vi "TEST_Menu.vi"() -> ()   [LabVIEW 2021, in "Menu.lvlib" / "Menu.lvclass"]
uses:
  Menu.lvclass
  <vilib>/Utility/miscctls.llb/LVMenuShortCut.ctl
  MenuSelection.ctl
  Picture2D/src/Color/Color.lvclass
  Picture2D/src/2DPictureControl/2DPictureControl.lvclass
  <vilib>/Utility/miscctls.llb/LVPointTypeDef.ctl
  91be992c-c2ba-4221-a176-dbd6ab68e1f9.vi
  Picture2D/src/Picture/Image.lvclass
  C:/GitHub/Picture2D/src/IDrawable/IDrawable.lvclass
  SetBackgroundColor.vi
  SetBorderColor.vi
  SetHiliteColor.vi
  SetHiliteTextColor.vi
  SetTextColor.vi
  <vilib>/ErrorRing/Error Ring.xnode
panel:
  out "enabled":bool
  out "2D Picture out":picture
  in  "Color Theme":enum16{"LabVIEW", "Dark"}(ring)
  out "item name":string
  out "submenu tags":string[](array[string])
  out "checked":bool
  out "short cut":T1
  out "2D Picture":picture
  out "ItemPath":string
  out "ItemTag":string
  out "error out":errorcluster
  out "item tags out":string[](array[string])
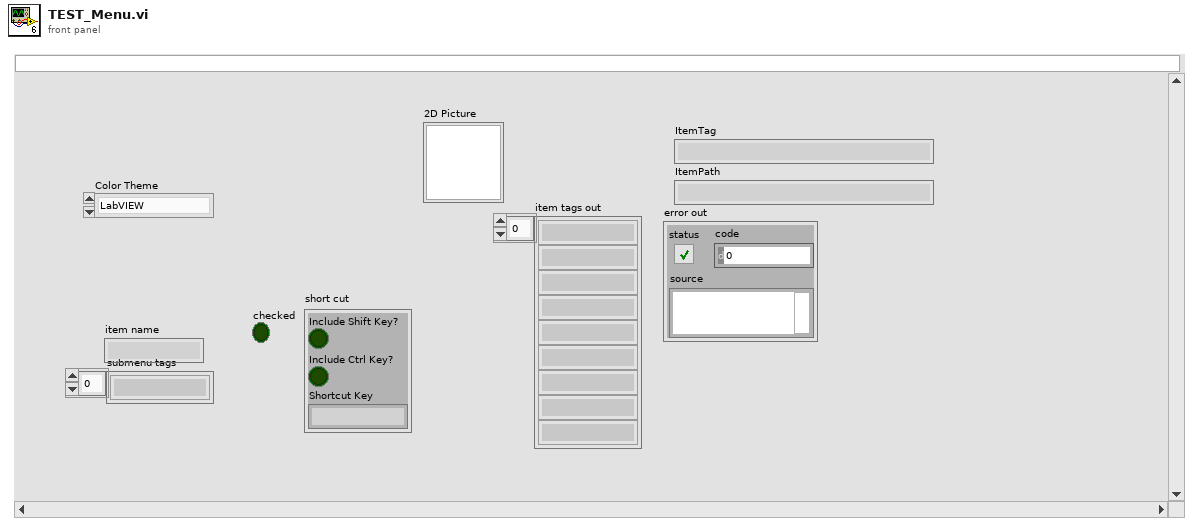
[diagram p1: front panel]
types:
  T1 = typedef "LVMenuShortCut.ctl" = cluster{"Include Shift Key?":bool, "Include Ctrl Key?":bool, "Shortcut Key":string}
  T2 = enum16{"Init Menu", "Init Menu Icon", "Execute", "Close"}
  T3 = enum16{"Init Menu", "Init Menu Icon", "Execute", "Close"}[]
  T4 = typedef "LVPointTypeDef.ctl" = cluster{"Horizontal":i16, "Vertical":i16}
  T5 = typedef "LVBoundsTypeDef.ctl" = cluster{"Width":u32, "Height":u32}
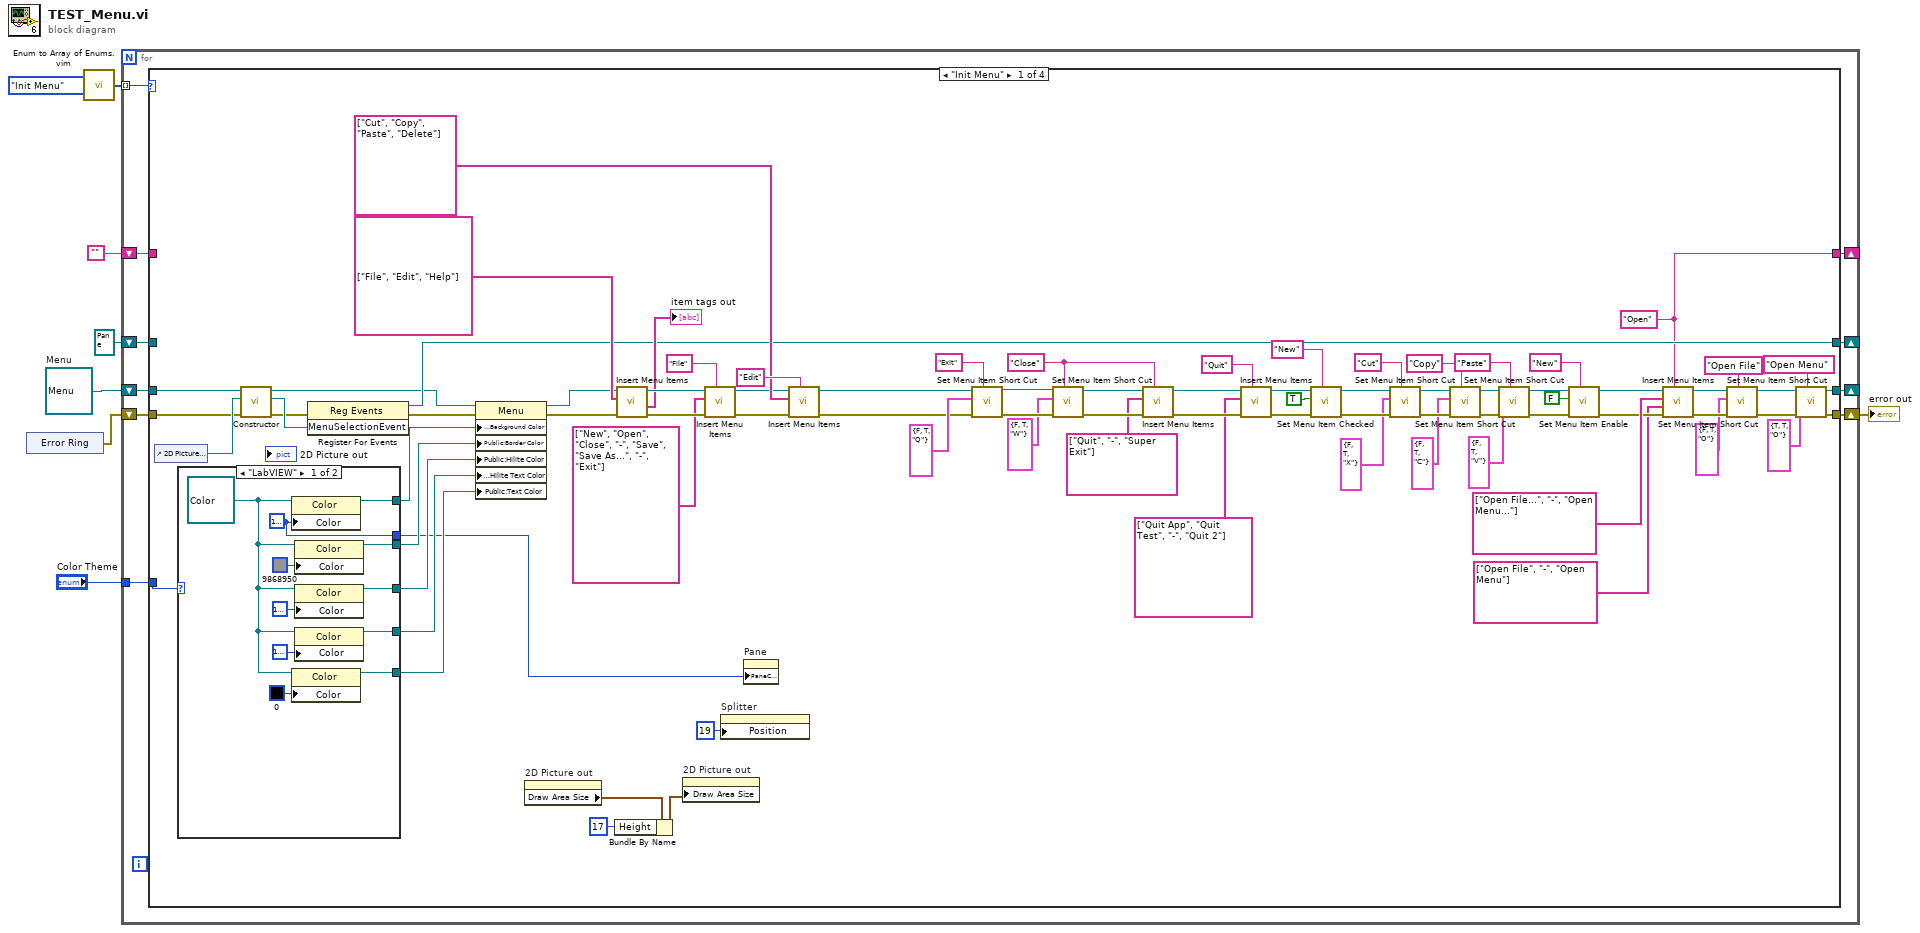
[diagram p0: block diagram]
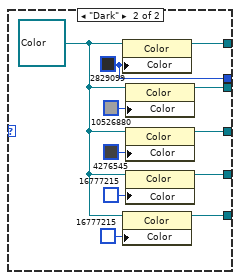
[diagram p2: hidden frame]
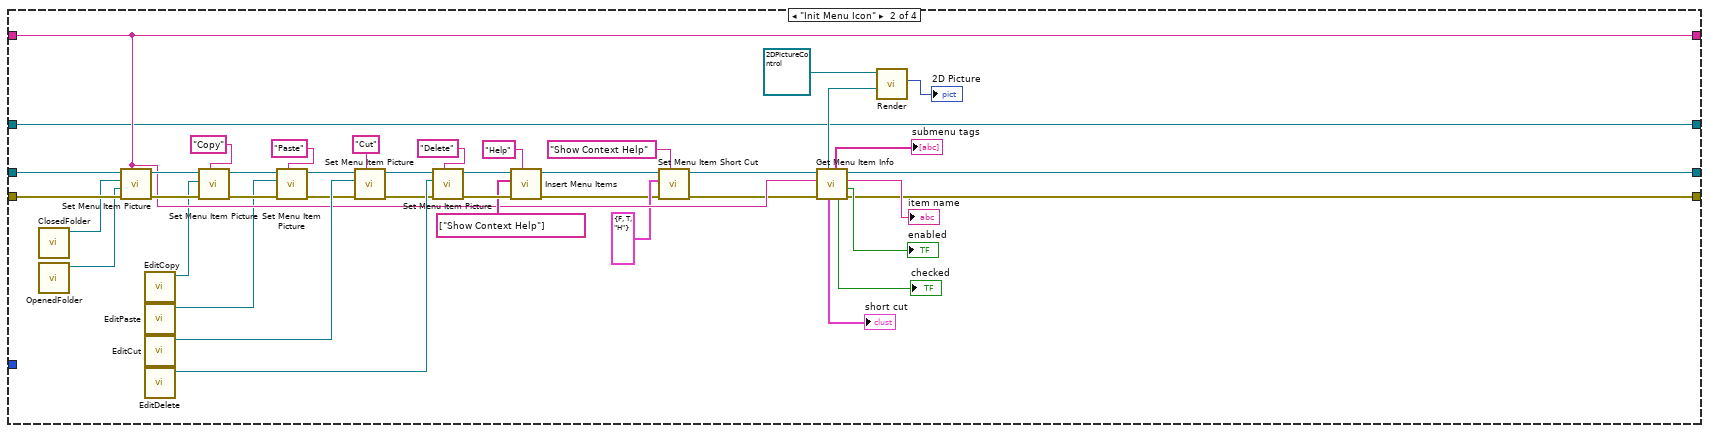
[diagram p3: hidden frame]
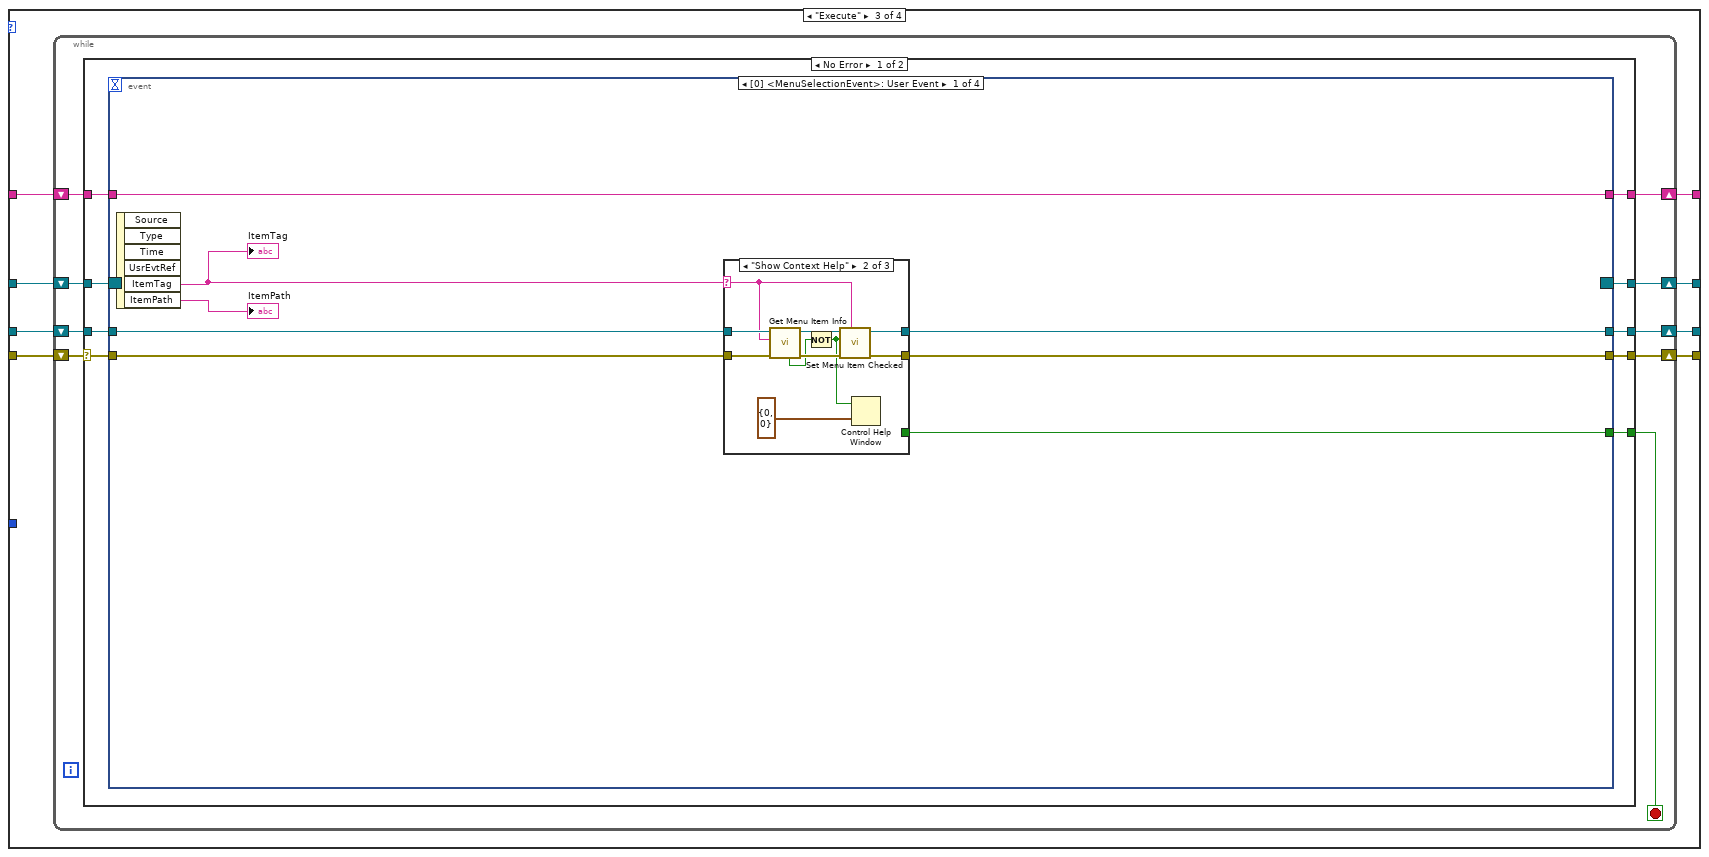
[diagram p4: hidden frame]
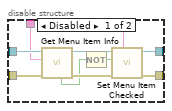
[diagram p6: hidden frame]
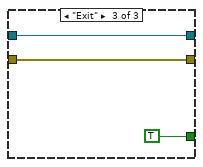
[diagram p7: hidden frame]
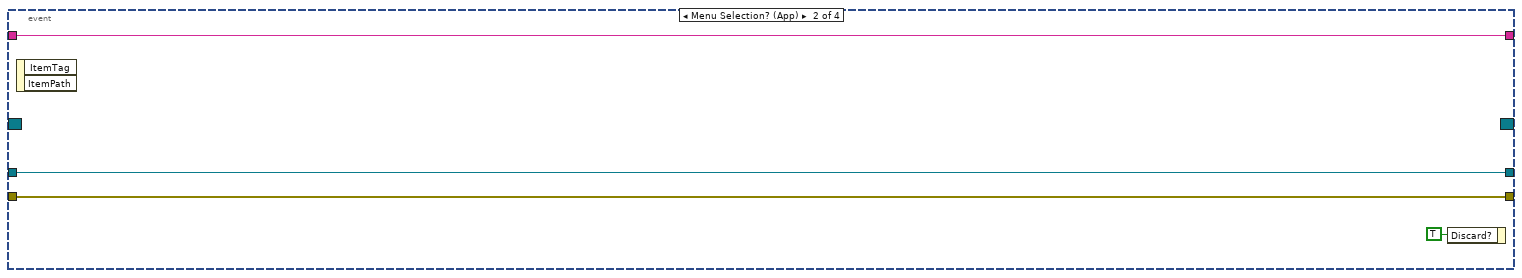
[diagram p8: hidden frame]
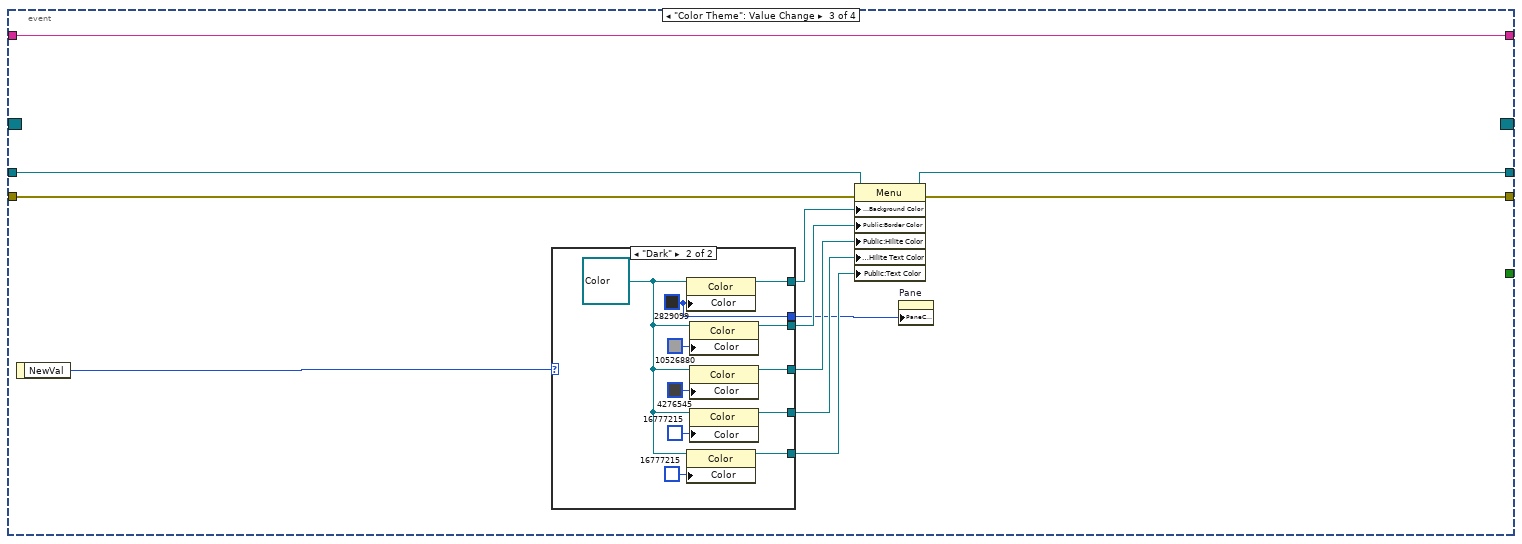
[diagram p9: hidden frame]
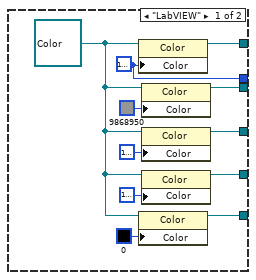
[diagram p10: hidden frame]
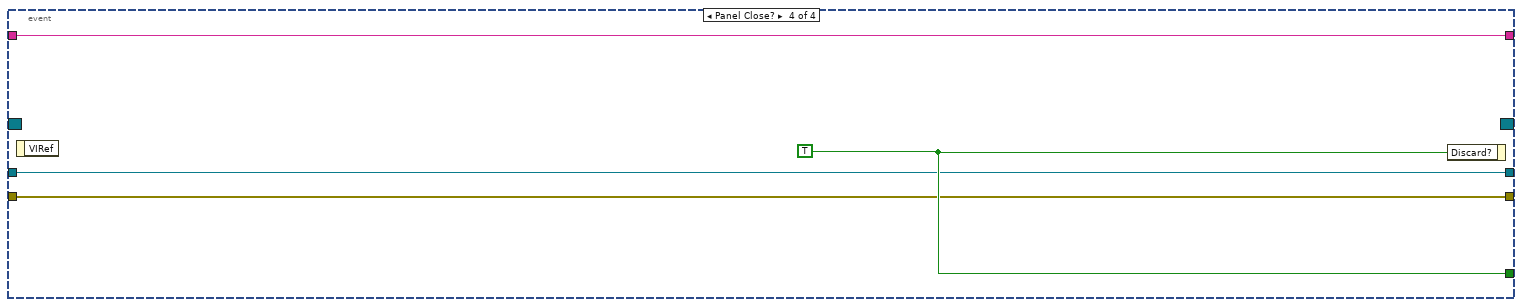
[diagram p11: hidden frame]
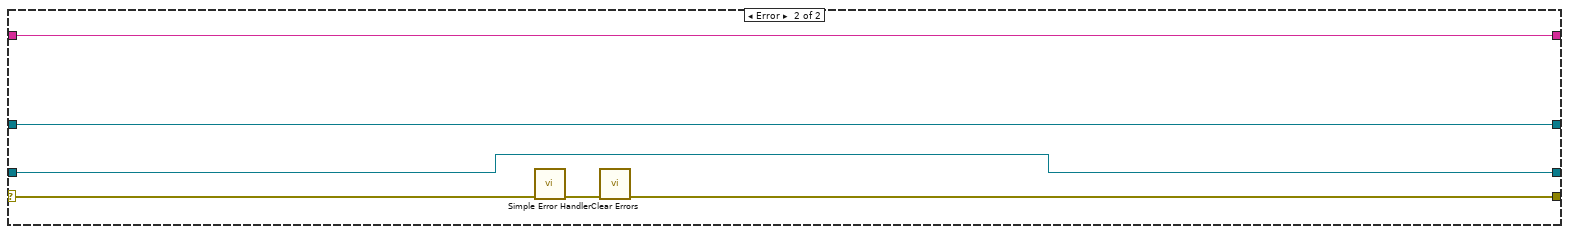
[diagram p12: hidden frame]
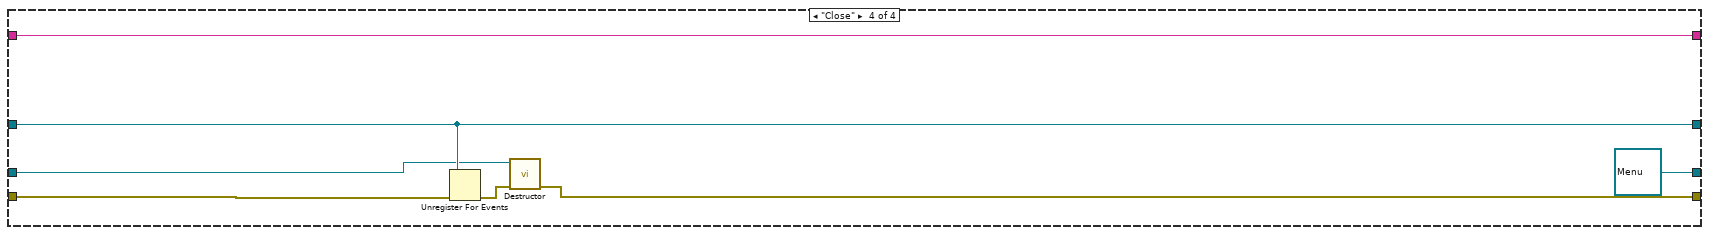
[diagram p13: hidden frame]
diagram:
  w8 = refnum<class "Menu.lvclass"> refnum  # Menu
  n1 = xnode "Error Ring"() -> ("error out"=w4:errorcluster)
  n2 = call "Enum to Array of Enums.vim"("enum"=T2."Init Menu") -> ("array of enums"=w5:T3)
  n3 = for {
    tunnel: "Color Theme" -> [w16]
    shift-right: [w15] -> _
    shift-left: w8 -> [w18]
    tunnel: w5 -> [w12] mode=indexing
    shift-right: [w14] -> w3
    shift-left: w4 -> [w13]
    shift-right: [w17] -> _
    shift-left: refnum<event-registration> refnum ("Event Registration Refnum") -> [w9]
    shift-right: [w11] -> _
    shift-left: "" -> [w10]
    n4 = case shown="\"Init Menu\"" w12 {
      tunnel: w18 -> [w99 w134 w169 w278]
      tunnel: [w74 w135 w170 w280] -> w17
      tunnel: [w68 w136 w164 w276] -> w11
      tunnel: w16 -> [w40 _ _ _]
      tunnel: [w33 w137 w168 refnum<class "Menu.lvclass"> refnum ("Menu")] -> w15
      tunnel: [w32 w138 w167 w279] -> w14
      tunnel: w13 -> [w26 w133 w166 w275]
      tunnel: w10 -> [_ w136 w165 w276]
      tunnel: w9 -> [_ w135 w171 w280]
      frame "Init Menu" {
        w68 = "Open" ("item tag")
        w81 = "Close" ("item tag")
        n5 = control-ref of="2D Picture out"() -> (w75:refnum<vi>)
        n6 = case shown="\"LabVIEW\"" w40 {
          tunnel: [w110 w121] -> w45
          tunnel: [w108 w119] -> w44
          tunnel: [w107 w118] -> w43
          tunnel: [w106 w117] -> w42
          tunnel: [w105 w116] -> w41
          tunnel: [w100 w111] -> w39
          frame "LabVIEW" {
            w100 = u32 16777238 ("Color")
            w109 = refnum<class "Color.lvclass"> refnum ("Background Color")
            n7 = property class="Color"(reference=w109, "Color"=w100) -> (reference out=w110:refnum<class "Color.lvclass">)  [unwired: 1 in, 1 out]
            n8 = property class="Color"(reference=w109, "Color"=u32 0) -> (reference out=w105:refnum<class "Color.lvclass">)  [unwired: 1 in, 1 out]
            n9 = property class="Color"(reference=w109, "Color"=u32 9868950) -> (reference out=w108:refnum<class "Color.lvclass">)  [unwired: 1 in, 1 out]
            n10 = property class="Color"(reference=w109, "Color"=u32 16777224) -> (reference out=w107:refnum<class "Color.lvclass">)  [unwired: 1 in, 1 out]
            n11 = property class="Color"(reference=w109, "Color"=u32 16777226) -> (reference out=w106:refnum<class "Color.lvclass">)  [unwired: 1 in, 1 out]
          }
          frame "Dark" {
            w111 = u32 2829099 ("Color")
            w120 = refnum<class "Color.lvclass"> refnum ("Background Color")
            n12 = property class="Color"(reference=w120, "Color"=w111) -> (reference out=w121:refnum<class "Color.lvclass">)  [unwired: 1 in, 1 out]
            n13 = property class="Color"(reference=w120, "Color"=u32 16777215) -> (reference out=w116:refnum<class "Color.lvclass">)  [unwired: 1 in, 1 out]
            n14 = property class="Color"(reference=w120, "Color"=u32 10526880) -> (reference out=w119:refnum<class "Color.lvclass">)  [unwired: 1 in, 1 out]
            n15 = property class="Color"(reference=w120, "Color"=u32 4276545) -> (reference out=w118:refnum<class "Color.lvclass">)  [unwired: 1 in, 1 out]
            n16 = property class="Color"(reference=w120, "Color"=u32 16777215) -> (reference out=w117:refnum<class "Color.lvclass">)  [unwired: 1 in, 1 out]
          }
        }
        n17 = call "Constructor.vi"("error in (no error)"=w26, "PictRef"=w75, "Menu in"=w99) -> ("error out"=w90:errorcluster, "MenuSelectionEvent"=w92:refnum<user-event>, "Menu out"=w47:refnum<class "Menu.lvclass">)  [unwired: 6 in]
        n18 = register-events(error in=w90, w92) -> (reference out=w74:refnum<event-registration>, error out=w91:errorcluster)  [unwired: 1 in]
        n19 = property class="Menu"(reference=w47, error in=w91, "Public:Background Color"=w45, "Public:Border Color"=w44, "Public:Hilite Color"=w43, "Public:Hilite Text Color"=w42, "Public:Text Color"=w41) -> (reference out=w46:refnum<class "Menu.lvclass">, error out=w48:errorcluster)
        n20 = property on="2D Picture out" class="Pict"() -> ("Draw Area Size"=w24:T5)  [unwired: 2 in, 2 out]
        n21 = Bundle By Name(cluster=w24, "Height"=u32 17) -> (w23:T5)
        n22 = call "Insert Menu Items.vi"("error in (no error)"=w48, "item names"=string[] ["File", "Edit", "Help"], "Menu in"=w46) -> ("error out"=w96:errorcluster, "item tags out"=→"item tags out":string[], "Menu out"=w97:refnum<class "Menu.lvclass">)  [unwired: 6 in]
        n23 = property on="2D Picture out" class="Pict"("Draw Area Size"=w23) -> ()  [unwired: 2 in, 2 out]
        n24 = call "Insert Menu Items.vi"("menu tag"="File", "error in (no error)"=w96, "item names"=string[] ["New", "Open", "Close", "-", "Save", "Save As...", "-", "Exit"], "Menu in"=w97) -> ("error out"=w49:errorcluster, "Menu out"=w50:refnum<class "Menu.lvclass">)  [unwired: 5 in, 1 out]
        n25 = property on="Splitter" class="Splitter"("Position"=19 ("Splitter Position")) -> ()  [unwired: 2 in, 2 out]
        n26 = property on="Pane" class="Pane"("PaneColor"=w39) -> ()  [unwired: 2 in, 2 out]
        n27 = call "Insert Menu Items.vi"("menu tag"="Edit", "error in (no error)"=w49, "item names"=string[] ["Cut", "Copy", "Paste", "Delete"], "Menu in"=w50) -> ("error out"=w21:errorcluster, "Menu out"=w20:refnum<class "Menu.lvclass">)  [unwired: 5 in, 1 out]
        n28 = call "Set Menu Item Short Cut.vi"("item tag"="Exit", "error in (no error)"=w21, "short cut"=T1 {"Include Shift Key?"=FALSE, "Include Ctrl Key?"=TRUE, "Shortcut Key"="Q"}, "Menu in"=w20) -> ("error out"=w86:errorcluster, "Menu out"=w85:refnum<class "Menu.lvclass">)  [unwired: 6 in]
        n29 = call "Set Menu Item Short Cut.vi"("item tag"=w81, "error in (no error)"=w86, "short cut"=T1 {"Include Shift Key?"=FALSE, "Include Ctrl Key?"=TRUE, "Shortcut Key"="W"}, "Menu in"=w85) -> ("error out"=w82:errorcluster, "Menu out"=w83:refnum<class "Menu.lvclass">)  [unwired: 6 in]
        n30 = call "Insert Menu Items.vi"("menu tag"=w81, "error in (no error)"=w82, "item names"=string[] ["Quit", "-", "Super Exit"], "Menu in"=w83) -> ("error out"=w78:errorcluster, "Menu out"=w77:refnum<class "Menu.lvclass">)  [unwired: 5 in, 1 out]
        n31 = call "Insert Menu Items.vi"("menu tag"="Quit", "error in (no error)"=w78, "item names"=string[] ["Quit App", "Quit Test", "-", "Quit 2"], "Menu in"=w77) -> ("error out"=w72:errorcluster, "Menu out"=w73:refnum<class "Menu.lvclass">)  [unwired: 5 in, 1 out]
        n32 = call "Set Menu Item Checked.vi"("item tag"="New", "error in (no error)"=w72, "checked"=TRUE, "Menu in"=w73) -> ("error out"=w66:errorcluster, "Menu out"=w67:refnum<class "Menu.lvclass">)  [unwired: 6 in]
        n33 = call "Set Menu Item Short Cut.vi"("item tag"="Cut", "error in (no error)"=w66, "short cut"=T1 {"Include Shift Key?"=FALSE, "Include Ctrl Key?"=TRUE, "Shortcut Key"="X"}, "Menu in"=w67) -> ("error out"=w63:errorcluster, "Menu out"=w62:refnum<class "Menu.lvclass">)  [unwired: 6 in]
        n34 = call "Set Menu Item Short Cut.vi"("item tag"="Copy", "error in (no error)"=w63, "short cut"=T1 {"Include Shift Key?"=FALSE, "Include Ctrl Key?"=TRUE, "Shortcut Key"="C"}, "Menu in"=w62) -> ("error out"=w65:errorcluster, "Menu out"=w64:refnum<class "Menu.lvclass">)  [unwired: 6 in]
        n35 = call "Set Menu Item Short Cut.vi"("item tag"="Paste", "error in (no error)"=w65, "short cut"=T1 {"Include Shift Key?"=FALSE, "Include Ctrl Key?"=TRUE, "Shortcut Key"="V"}, "Menu in"=w64) -> ("error out"=w56:errorcluster, "Menu out"=w54:refnum<class "Menu.lvclass">)  [unwired: 6 in]
        n36 = call "Set Menu Item Enable.vi"("item tag"="New", "error in (no error)"=w56, "enabled"=FALSE, "Menu in"=w54) -> ("error out"=w55:errorcluster, "Menu out"=w53:refnum<class "Menu.lvclass">)  [unwired: 6 in]
        n37 = call "Insert Menu Items.vi"("menu tag"=w68, "error in (no error)"=w55, "item tags"=string[] ["Open File", "-", "Open Menu"] ("item names"), "item names"=string[] ["Open File...", "-", "Open Menu..."], "Menu in"=w53) -> ("error out"=w36:errorcluster, "Menu out"=w37:refnum<class "Menu.lvclass">)  [unwired: 4 in, 1 out]
        n38 = call "Set Menu Item Short Cut.vi"("item tag"="Open File", "error in (no error)"=w36, "short cut"=T1 {"Include Shift Key?"=FALSE, "Include Ctrl Key?"=TRUE, "Shortcut Key"="O"}, "Menu in"=w37) -> ("error out"=w35:errorcluster, "Menu out"=w34:refnum<class "Menu.lvclass">)  [unwired: 6 in]
        n39 = call "Set Menu Item Short Cut.vi"("item tag"="Open Menu", "error in (no error)"=w35, "short cut"=T1 {"Include Shift Key?"=TRUE, "Include Ctrl Key?"=TRUE, "Shortcut Key"="O"}, "Menu in"=w34) -> ("error out"=w32:errorcluster, "Menu out"=w33:refnum<class "Menu.lvclass">)  [unwired: 6 in]
      }
      frame "Init Menu Icon" {
        n40 = call "ClosedFolder.vi"() -> ("Image out"=w123:refnum<class "Image.lvclass">)  [unwired: 11 in]
        n41 = call "OpenedFolder.vi"() -> ("Image out"=w122:refnum<class "Image.lvclass">)  [unwired: 11 in]
        n42 = call "Set Menu Item Picture.vi"("item tag"=w136, "error in (no error)"=w133, "Hilite Picture"=w122, "Picture"=w123, "Menu in"=w134) -> ("error out"=w153:errorcluster, "Menu out"=w152:refnum<class "Menu.lvclass">)  [unwired: 5 in]
        n43 = call "EditCopy.vi"() -> ("Image out"=w125:refnum<class "Image.lvclass">)  [unwired: 11 in]
        n44 = call "EditPaste.vi"() -> ("Image out"=w124:refnum<class "Image.lvclass">)  [unwired: 11 in]
        n45 = call "EditCut.vi"() -> ("Image out"=w162:refnum<class "Image.lvclass">)  [unwired: 11 in]
        n46 = call "EditDelete.vi"() -> ("Image out"=w163:refnum<class "Image.lvclass">)  [unwired: 11 in]
        n47 = call "Set Menu Item Picture.vi"("item tag"="Copy", "error in (no error)"=w153, "Picture"=w125, "Menu in"=w152) -> ("error out"=w155:errorcluster, "Menu out"=w154:refnum<class "Menu.lvclass">)  [unwired: 6 in]
        n48 = call "Set Menu Item Picture.vi"("item tag"="Paste", "error in (no error)"=w155, "Picture"=w124, "Menu in"=w154) -> ("error out"=w157:errorcluster, "Menu out"=w156:refnum<class "Menu.lvclass">)  [unwired: 6 in]
        n49 = call "Set Menu Item Picture.vi"("item tag"="Cut", "error in (no error)"=w157, "Picture"=w162, "Menu in"=w156) -> ("error out"=w159:errorcluster, "Menu out"=w158:refnum<class "Menu.lvclass">)  [unwired: 6 in]
        n50 = call "Set Menu Item Picture.vi"("item tag"="Delete", "error in (no error)"=w159, "Picture"=w163, "Menu in"=w158) -> ("error out"=w161:errorcluster, "Menu out"=w160:refnum<class "Menu.lvclass">)  [unwired: 6 in]
        n51 = call "Insert Menu Items.vi"("menu tag"="Help", "error in (no error)"=w161, "item names"=string[] ["Show Context Help"], "Menu in"=w160) -> ("error out"=w131:errorcluster, "Menu out"=w129:refnum<class "Menu.lvclass">)  [unwired: 5 in, 1 out]
        n52 = call "Set Menu Item Short Cut.vi"("item tag"="Show Context Help", "error in (no error)"=w131, "short cut"=T1 {"Include Shift Key?"=FALSE, "Include Ctrl Key?"=TRUE, "Shortcut Key"="H"}, "Menu in"=w129) -> ("error out"=w130:errorcluster, "Menu out"=w128:refnum<class "Menu.lvclass">)  [unwired: 6 in]
        n53 = call "Get Menu Item Info.vi"("error in (no error)"=w130, "item tag"=w136, "Menu in"=w128) -> ("error out"=w138:errorcluster, "enabled"=→"enabled":bool, "item name"=→"item name":string, "Menu out"=w137:refnum<class "Menu.lvclass">, "checked"=→"checked":bool, "submenu tags"=→"submenu tags":string[], "short cut"=→"short cut":T1, "Picture"=w140:refnum<class "Image.lvclass">)  [unwired: 1 in]
        n54 = call-dynamic "Render.vi"("IDrawable"=w140, "2DPictureControl in"=refnum<class "2DPictureControl.lvclass"> refnum) -> ("2D Picture out"=→"2D Picture":picture)  [unwired: 7 in, 2 out]
      }
      frame "Execute" {
        n55 = while {
          shift-right: [w178] -> w167
          shift-left: w166 -> [w179]
          shift-right: [w175] -> w170
          shift-left: w171 -> [w180]
          shift-right: [w176] -> w168
          shift-left: w169 -> [w177]
          shift-right: [w172] -> w164
          shift-left: w165 -> [w173]
          stop <- w174 stop-if-true
          n56 = case shown="No Error" w179 {
            selector: w179 -> [w188 w274]
            tunnel: w180 -> [w189 w273]
            tunnel: [w187 w270] -> w178
            tunnel: w177 -> [w186 w272]
            tunnel: [w185 w272] -> w176
            tunnel: [w184 w273] -> w175
            tunnel: [w183 _] -> w174
            tunnel: w173 -> [w182 w269]
            tunnel: [w181 w269] -> w172
            frame No Error {
              n57 = event shown="[0] <MenuSelectionEvent>: User Event" {
                selector: w189 -> [_ _ _ _]
                dyn-events: [_ _ _ _] -> w184
                timeout: _ -> [_ _ _ _]
                tunnel: [w192 w230 w233 w267] -> w187
                tunnel: w188 -> [w193 w230 w236 w267]
                tunnel: [w191 w229 w232 w266] -> w185
                tunnel: w186 -> [w194 w229 w235 w266]
                tunnel: [w195 _ _ w268] -> w183
                tunnel: w182 -> [w190 w228 w231 w265]
                tunnel: [w190 w228 w231 w265] -> w181
                event User Event {
                  n58 = event-data() -> ("ItemTag"=w196:string, "ItemPath"=→"ItemPath":string)  [unwired: 1 in, 4 out]
                  "ItemTag" <- w196
                  n59 = case shown="\"Show Context Help\"" w196 {
                    selector: w196 -> [w198 w217 _]
                    tunnel: [_ _ TRUE] -> w195
                    tunnel: w194 -> [w202 w223 w225]
                    tunnel: w193 -> [w201 w222 w224]
                    tunnel: [w200 w220 w224] -> w192
                    tunnel: [w199 w218 w225] -> w191
                    frame Default {
                      n60 = disable-structure shown="Enabled" {
                        disable-tunnel: w202 -> [w211 w213]
                        disable-tunnel: w201 -> [w210 w212]
                        disable-tunnel: [w208 w212] -> w200
                        disable-tunnel: [w206 w213] -> w199
                        disable-tunnel: w198 -> [w203 _]
                        frame Disabled {
                          n61 = call "Get Menu Item Info.vi"("error in (no error)"=w210, "item tag"=w203, "Menu in"=w211) -> ("error out"=w209:errorcluster, "Menu out"=w207:refnum<class "Menu.lvclass">, "checked"=w205:bool)  [unwired: 1 in, 5 out]
                          n62 = Not(x=w205) -> (.not. x?=w204:bool)
                          n63 = call "Set Menu Item Checked.vi"("item tag"=w203, "error in (no error)"=w209, "checked"=w204, "Menu in"=w207) -> ("error out"=w208:errorcluster, "Menu out"=w206:refnum<class "Menu.lvclass">)  [unwired: 6 in]
                        }
                        frame Enabled {
                        }
                      }
                    }
                    frame "Show Context Help" {
                      n64 = call "Get Menu Item Info.vi"("error in (no error)"=w222, "item tag"=w217, "Menu in"=w223) -> ("error out"=w221:errorcluster, "Menu out"=w219:refnum<class "Menu.lvclass">, "checked"=w215:bool)  [unwired: 1 in, 5 out]
                      n65 = Not(x=w215) -> (.not. x?=w214:bool)
                      n66 = call "Set Menu Item Checked.vi"("item tag"=w217, "error in (no error)"=w221, "checked"=w214, "Menu in"=w219) -> ("error out"=w220:errorcluster, "Menu out"=w218:refnum<class "Menu.lvclass">)  [unwired: 6 in]
                      n67 = Control Help Window(0:T4 {"Horizontal"=0, "Vertical"=0} ("Top Left Corner"), 1:w214) -> ()
                    }
                    frame "Exit" {
                    }
                  }
                }
                event Menu Selection? (App) {
                  n68 = event-data() -> ()  [unwired: 1 in, 2 out]
                  n69 = event-data("Discard?"=TRUE) -> ()  [unwired: 1 in, 1 out]
                }
                event "Color Theme": Value Change {
                  n70 = event-data() -> ("NewVal"=w237:enum16{"LabVIEW", "Dark"})  [unwired: 1 in]
                  n71 = case shown="\"Dark\"" w237 {
                    tunnel: [w253 w264] -> w242
                    tunnel: [w251 w262] -> w241
                    tunnel: [w250 w261] -> w240
                    tunnel: [w249 w260] -> w239
                    tunnel: [w248 w259] -> w238
                    tunnel: [w243 w254] -> w234
                    frame "LabVIEW" {
                      w243 = u32 16777238 ("Color")
                      w252 = refnum<class "Color.lvclass"> refnum ("Background Color")
                      n72 = property class="Color"(reference=w252, "Color"=w243) -> (reference out=w253:refnum<class "Color.lvclass">)  [unwired: 1 in, 1 out]
                      n73 = property class="Color"(reference=w252, "Color"=u32 0) -> (reference out=w248:refnum<class "Color.lvclass">)  [unwired: 1 in, 1 out]
                      n74 = property class="Color"(reference=w252, "Color"=u32 9868950) -> (reference out=w251:refnum<class "Color.lvclass">)  [unwired: 1 in, 1 out]
                      n75 = property class="Color"(reference=w252, "Color"=u32 16777224) -> (reference out=w250:refnum<class "Color.lvclass">)  [unwired: 1 in, 1 out]
                      n76 = property class="Color"(reference=w252, "Color"=u32 16777226) -> (reference out=w249:refnum<class "Color.lvclass">)  [unwired: 1 in, 1 out]
                    }
                    frame "Dark" {
                      w254 = u32 2829099 ("Color")
                      w263 = refnum<class "Color.lvclass"> refnum ("Background Color")
                      n77 = property class="Color"(reference=w263, "Color"=w254) -> (reference out=w264:refnum<class "Color.lvclass">)  [unwired: 1 in, 1 out]
                      n78 = property class="Color"(reference=w263, "Color"=u32 16777215) -> (reference out=w259:refnum<class "Color.lvclass">)  [unwired: 1 in, 1 out]
                      n79 = property class="Color"(reference=w263, "Color"=u32 10526880) -> (reference out=w262:refnum<class "Color.lvclass">)  [unwired: 1 in, 1 out]
                      n80 = property class="Color"(reference=w263, "Color"=u32 4276545) -> (reference out=w261:refnum<class "Color.lvclass">)  [unwired: 1 in, 1 out]
                      n81 = property class="Color"(reference=w263, "Color"=u32 16777215) -> (reference out=w260:refnum<class "Color.lvclass">)  [unwired: 1 in, 1 out]
                    }
                  }
                  n82 = property class="Menu"(reference=w235, error in=w236, "Public:Background Color"=w242, "Public:Border Color"=w241, "Public:Hilite Color"=w240, "Public:Hilite Text Color"=w239, "Public:Text Color"=w238) -> (reference out=w232:refnum<class "Menu.lvclass">, error out=w233:errorcluster)
                  n83 = property on="Pane" class="Pane"("PaneColor"=w234) -> ()  [unwired: 2 in, 2 out]
                }
                event Panel Close? {
                  w268 = TRUE ("Discard?")
                  n84 = event-data() -> ()  [unwired: 1 in, 1 out]
                  n85 = event-data("Discard?"=w268) -> ()  [unwired: 1 in, 1 out]
                }
              }
            }
            frame Error {
              n86 = call <vilib>:"Simple Error Handler.vi"("error in (no error)"=w274) -> ("error out"=w271:errorcluster)  [unwired: 4 in, 4 out]
              n87 = call <vilib>:"Clear Errors.vi"("error in (no error)"=w271) -> ("error out"=w270:errorcluster)  [unwired: 5 in, 1 out]
            }
          }
        }
      }
      frame "Close" {
        n88 = Unregister For Events(event registration refnum=w280, error in=w275) -> (error out=w281:errorcluster)
        n89 = call "Destructor.vi"("error in (no error)"=w281, "Menu in"=w278) -> ("error out"=w279:errorcluster)  [unwired: 9 in]
      }
    }
  }
  "error out" <- w3
